vi "Show Head Point.vi"(8 "error in (no error)":errorcluster, 9 "XY Plot":refnum<vi>, 10 "DataSet":T1(array[cluster])) -> (0 "error out":errorcluster, 1 "XY Plot out":refnum<vi>, 3 "picture out":picture)   [LabVIEW 2025, in "XY Plotter.lvlib" / "XY Plotter.lvclass"]
uses:
  XY Plotter.lvclass
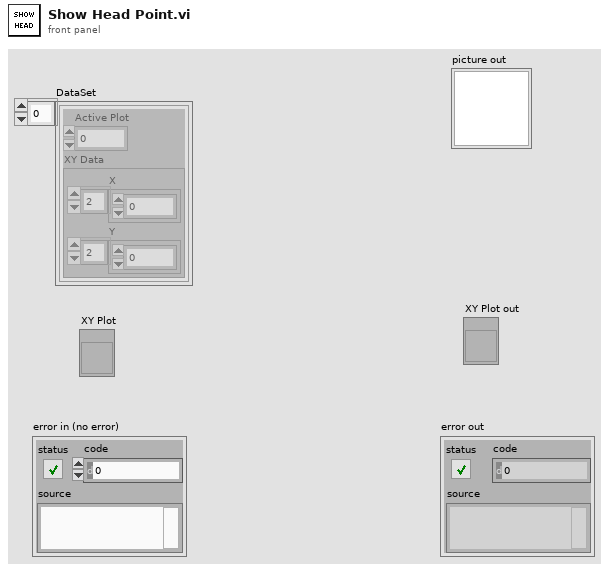
[diagram p1: front panel]
types:
  T1 = cluster{"Active Plot":u32, "XY Data":cluster{"X":dbl[], "Y":dbl[]}}[]
  T2 = typedef "LVRectTypeDef.ctl" = cluster{"Left":i16, "Top":i16, "Right":i16, "Bottom":i16}
  T3 = typedef "LVPoint32TypeDef.ctl" = cluster{"Horizontal":i32, "Vertical":i32}
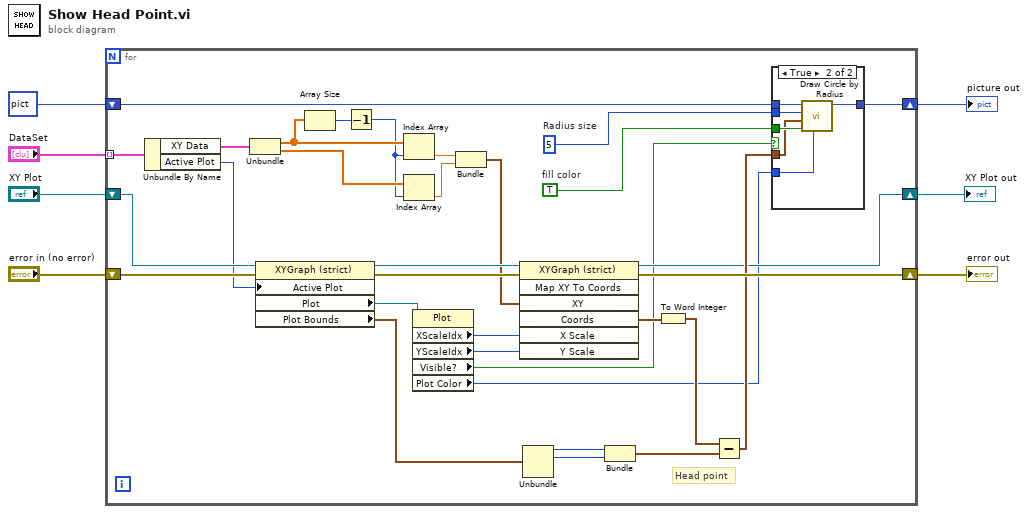
[diagram p0: block diagram]
diagram:
  n1 = for {
    tunnel: "DataSet" -> [w12] mode=indexing
    shift-right: [w15] -> w5
    shift-left: "XY Plot" -> [w39]
    shift-right: [w31] -> w6
    shift-left: "error in (no error)" -> [w38]
    shift-right: [w37] -> w3
    shift-left: picture data[5B] ("Plot Images:Front") -> [w18]
    w19 = i16 5  # Radius size
    w36 = TRUE  # fill color
    # "Head point"
    n2 = Unbundle By Name(w12) -> ("XY Data"=w10:cluster{"X":dbl[], "Y":dbl[]}, "Active Plot"=w11:u32)
    n3 = Unbundle(w10) -> ("X"=w17:dbl[], "Y"=w25:dbl[])
    n4 = property class="XYGraph (strict)"(reference=w39, error in=w38, "Active Plot"=w11) -> (reference out=w30:refnum<vi>, error out=w32:errorcluster, "Plot"=w35:refnum<vi>, "Plot Bounds"=w13:T2)
    n5 = Array Size(array=w17) -> (size(s)=w16:i32)
    n6 = Decrement(x=w16) -> (x-1=w14:i32)
    n7 = Index Array(array=w17, index=w14) -> (element=w24:dbl)
    n8 = Index Array(array=w25, index=w14) -> (element=w23:dbl)
    n9 = property class="Plot"(reference=w35) -> ("XScaleIdx"=w27:u32, "YScaleIdx"=w26:u32, "Visible?"=w9:bool, "Plot Color"=w8:u32)  [unwired: 1 in, 2 out]
    n10 = Bundle(w24, w23) -> (w22:cluster{dbl, dbl})  [unwired: 1 in]
    n11 = invoke on="Invoke Node" class="XYGraph (strict)" method="Map XY To Coords"(reference=w30, error in=w32, "XY"=w22, "X Scale"=w27, "Y Scale"=w26) -> (reference out=w15:refnum<vi>, error out=w31:errorcluster, "Coords"=w28:T3)  [unwired: 2 in, 4 out]
    n12 = Unbundle(w13) -> ("Left"=w34:i16, "Top"=w33:i16)  [unwired: 2 out]
    n13 = Bundle("Left"=w34, "Top"=w33) -> (w20:cluster{"Left":i16, "Top":i16})  [unwired: 1 in]
    n14 = To Word Integer(number=w28) -> (16bit integer=w21:cluster{"Horizontal":i16, "Vertical":i16})
    n15 = Subtract(x=w21, y=w20) -> (x-y=w29:cluster{i16, i16})
    n16 = case shown="True" w9 {
      tunnel: [w40 w46] -> w37
      tunnel: w36 -> [_ w45]
      tunnel: w29 -> [_ w44]
      tunnel: w19 -> [_ w43]
      tunnel: w18 -> [w40 w42]
      tunnel: w8 -> [_ w41]
      frame False {
      }
      frame True {
        n17 = call <vilib>:"Draw Circle by Radius.vi"("color(black)"=w41, "fill?(F)"=w45, "pixel center"=w44, "radius"=w43, "picture"=w42) -> ("new picture"=w46:picture)  [unwired: 6 in]
      }
    }
  }
  "error out" <- w6
  "picture out" <- w3
  "XY Plot out" <- w5
